vi "Write reference.vi"(8 "error in (no error)":errorcluster, 10 "reference":refnum<k24>, 11 "ToastService in":refnum<class "ToastService.lvclass">) -> (0 "error out":errorcluster, 3 "ToastService out":refnum<class "ToastService.lvclass">)   [LabVIEW 2026, in "ToastNotification.lvlib" / "ToastService.lvclass"]
doc: "Native data-member write accessor for the service notification manager reference. Store the supplied native handle without closing a previous handle or cloning the new one. The owning lifecycle method must release replaced resources. Pass the class and error through."
uses:
  ToastService.lvclass
  C:/Users/loicw/Documents/LabVIEW/ToastNotifications/Sources/bins/Microsoft.Toolkit.Uwp.Notifications.dll
  bins/Microsoft.Toolkit.Uwp.Notifications.dll
  ToastService.lvclass/ToastService.ctl
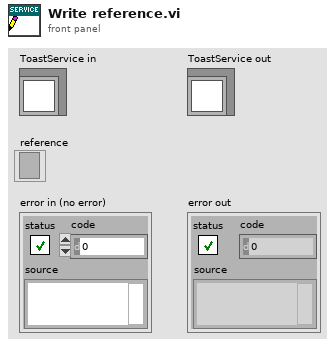
[diagram p1: front panel]
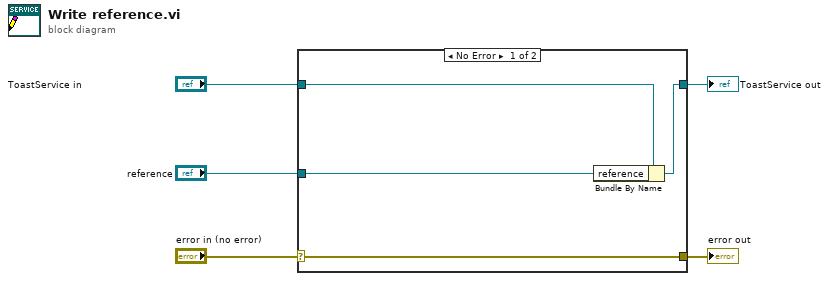
[diagram p0: block diagram]
diagram:
  n1 = case shown="No Error" "error in (no error)" {
    selector: "error in (no error)" -> [w9 w10]
    tunnel: [w9 w10] -> w4
    tunnel: [w7 w11] -> w2
    tunnel: "ToastService in" -> [w8 w11]
    tunnel: "reference" -> [w6 _]
    frame No Error {
      n2 = Bundle By Name(cluster=w8, "reference"=w6) -> (w7:refnum<class "ToastService.lvclass">)
    }
    frame Error {
    }
  }
  "error out" <- w4
  "ToastService out" <- w2
